vi "Launch in IDE.vi"() -> ()   [LabVIEW 2026]
uses:
  Actors/Runner/Runner/Runner.lvclass
  Actors/UI Logger/UI Logger.lvclass
  <vilib>/ActorFramework/Actor/Actor.lvclass
  Interfaces/IRunner/IRunner Messages/Run Msg/Run Msg.lvclass
  Interfaces/IRunner/IRunner Messages/Set Interfaces Msg/Set Interfaces Msg.lvclass
  <vilib>/AppBuilder/AB_API_Simple/Build Specification Version.ctl
  <vilib>/AppBuilder/AB_API_Simple/NI_App_Builder_API.lvlib
  Interfaces/ILogger Client/ILogger Client Messages/Set Logger Enqueuer Msg/Set Logger Enqueuer Msg.lvclass
panel:
  in  "Python Module":path
  in  "Output Folder":path
  # "py2vi direct Launcher"
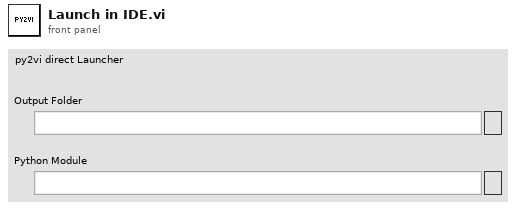
[diagram p1: front panel]
types:
  T1 = typedef "NI_App_Builder_API.lvlib/Build Specification Version.ctl" = cluster{"Major":u16, "Minor":u16, "Fix":u16, "Build":u16}
  T2 = typedef "IRunner.lvlib/IRunner.lvclass/Interfaces--cluster.ctl" = cluster{"IProject Manager":refnum<class "IProject Manager.lvclass">, "IFile Manager":refnum<class "IFile Manager.lvclass">, "IPython Caller":refnum<class "IPython Caller.lvclass">, "IElement Manager":refnum<class "IElement Manager.lvclass">, "ILV File Creator":refnum<class "ILV File Creator.lvclass">, "IHash Whitelist Handler":refnum<class "IHash Whitelist Handler.lvclass">}
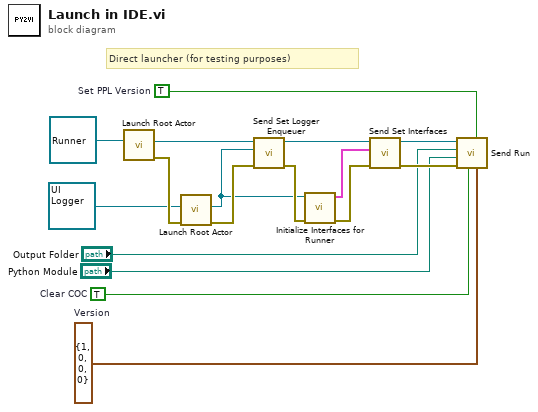
[diagram p0: block diagram]
diagram:
  w1 = TRUE  # Set PPL Version
  w13 = TRUE  # Clear COC
  w2 = T1 {"Major"=1, "Minor"=0, "Fix"=0, "Build"=0}  # Version
  # "Direct launcher (for testing purposes)"
  n1 = call <vilib>:"Launch Root Actor.vi"("Actor"=refnum<class "Runner.lvclass"> refnum ("G-CLI Runner.lvlib:G-CLI Runner.lvclass")) -> ("error out"=w8:errorcluster, "Actor's Enqueuer"=w11:refnum<class "Message Enqueuer.lvclass">)  [unwired: 9 in]
  n2 = call <vilib>:"Launch Root Actor.vi"("error in (no error)"=w8, "Actor"=refnum<class "UI Logger.lvclass"> refnum ("UI Logger.lvlib:UI Logger.lvclass")) -> ("error out"=w7:errorcluster, "Actor's Enqueuer"=w3:refnum<class "Message Enqueuer.lvclass">)  [unwired: 8 in]
  n3 = call "Send Set Logger Enqueuer.vi"("error in (no error)"=w7, "Logger"=w3, "Message Enqueuer"=w11) -> ("error out"=w9:errorcluster, "Message Enqueuer out"=w10:refnum<class "Message Enqueuer.lvclass">)  [unwired: 7 in]
  n4 = call "Initialize Interfaces for Runner.vi"("error in"=w9, "Logger Enqueuer"=w3) -> ("error out"=w16:errorcluster, "Interfaces"=w15:T2)  [unwired: 8 in]
  n5 = call "Send Set Interfaces.vi"("error in (no error)"=w16, "Interfaces"=w15, "Message Enqueuer"=w10) -> ("error out"=w14:errorcluster, "Message Enqueuer out"=w17:refnum<class "Message Enqueuer.lvclass">)  [unwired: 7 in]
  n6 = call "Send Run.vi"("Build Specification Version"=w2, "Set PPL Version"=w1, "Clear Compiled Object Cache"=w13, "error in (no error)"=w14, "Python Module"="Python Module", "Output Folder"="Output Folder", "Message Enqueuer"=w17) -> ()  [unwired: 3 in, 2 out]
